vi "PAQmem_constructor.vi"(8 "error in (no error)":errorcluster, 9 "TAGs":string[](array[string]), 10 "LayerInfo":T1, 11 "PAQ-memory in":refnum<class "PAQ-memory.lvclass">) -> (0 "error out":errorcluster, 3 "PAQ-memory out":refnum<class "PAQ-memory.lvclass">)   [LabVIEW 2020, in "Sgraph_lib_V1.lvlib" / "PAQ-memory.lvclass"]
uses:
  PAQ-memory.lvclass
  PAQ-memory.lvclass/PAQ-memory.ctl
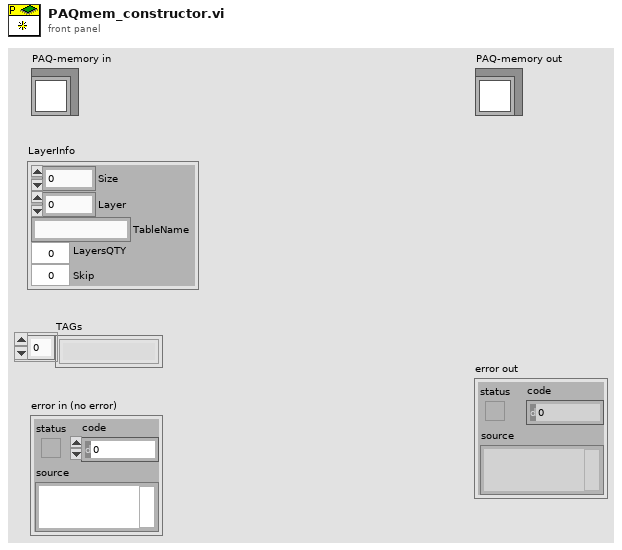
[diagram p1: front panel]
types:
  T1 = cluster{"Size":i32, "Layer":i32, "TableName":string, "LayersQTY":i32, "Skip":i32}
  T2 = cluster{"source":refnum<data-value>, "status":refnum<data-value>, "data":refnum<data-value>, "max":refnum<data-value>, "min":refnum<data-value>}
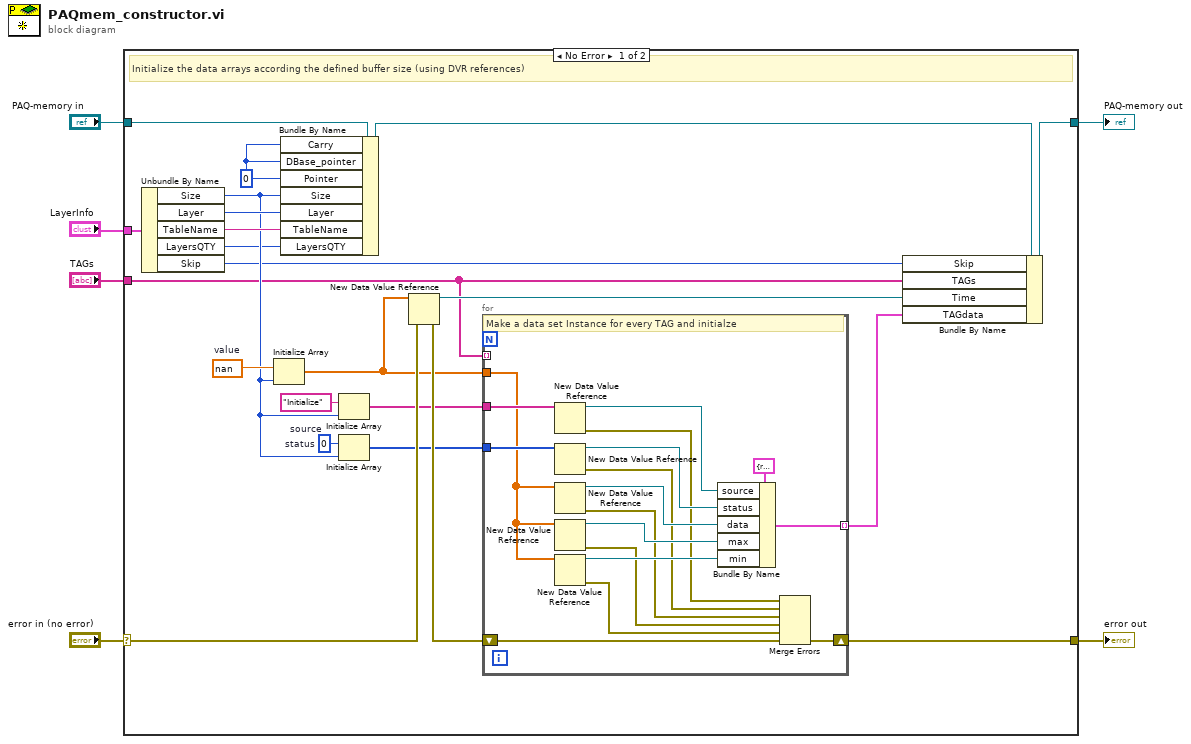
[diagram p0: block diagram]
diagram:
  n1 = case shown="No Error" "error in (no error)" {
    selector: "error in (no error)" -> [w18 w47]
    tunnel: [w15 w47] -> w1
    tunnel: [w19 w46] -> w2
    tunnel: "PAQ-memory in" -> [w25 w46]
    tunnel: "LayerInfo" -> [w28 _]
    tunnel: "TAGs" -> [w14 _]
    frame No Error {
      w21 = nan  # value
      w22 = u32 0  # status
      w23 = "Initialize"  # source
      w8 = 0 ("Pointer")
      # "Initialize the data arrays according the defined buffer size (using DVR references)"
      n2 = Unbundle By Name(w28) -> ("Size"=w17:i32, "Layer"=w27:i32, "TableName"=w26:string, "LayersQTY"=w13:i32, "Skip"=w7:i32)
      n3 = Initialize Array(w21, w17) -> (w12:dbl[])
      n4 = Bundle By Name(cluster=w25, "Carry"=w8, "DBase_pointer"=w8, "Pointer"=w8, "Size"=w17, "Layer"=w27, "TableName"=w26, "LayersQTY"=w13) -> (w24:refnum<class "PAQ-memory.lvclass">)
      n5 = Initialize Array(w23, w17) -> (w11:string[])
      n6 = Initialize Array(w22, w17) -> (w9:u32[])
      n7 = New Data Value Reference(data value=w12, error in=w18) -> (data value reference=w20:refnum<data-value>, error out=w16:errorcluster)
      n8 = for {
        tunnel: w12 -> [w38]
        tunnel: w11 -> [w40]
        shift-right: [w29] -> w15
        shift-left: w16 -> [w30]
        tunnel: w9 -> [w39]
        tunnel: [w36] -> w10 mode=indexing
        tunnel: w14 -> [_] mode=indexing
        # "Make a data set Instance for every TAG and initialze"
        n9 = New Data Value Reference(data value=w40) -> (data value reference=w45:refnum<data-value>, error out=w35:errorcluster)  [unwired: 1 in]
        n10 = New Data Value Reference(data value=w39) -> (data value reference=w44:refnum<data-value>, error out=w34:errorcluster)  [unwired: 1 in]
        n11 = New Data Value Reference(data value=w38) -> (data value reference=w43:refnum<data-value>, error out=w33:errorcluster)  [unwired: 1 in]
        n12 = New Data Value Reference(data value=w38) -> (data value reference=w42:refnum<data-value>, error out=w32:errorcluster)  [unwired: 1 in]
        n13 = New Data Value Reference(data value=w38) -> (data value reference=w41:refnum<data-value>, error out=w31:errorcluster)  [unwired: 1 in]
        n14 = Bundle By Name(cluster=T2 {"source"=refnum, "status"=refnum, "data"=refnum, "max"=refnum, "min"=refnum} ("TAGdata"), "source"=w45, "status"=w44, "data"=w43, "max"=w42, "min"=w41) -> (w36:T2)
        n15 = Merge Errors(w35, w34, w33, w32, w31, w30) -> (w29:errorcluster)
      }
      n16 = Bundle By Name(cluster=w24, "Skip"=w7, "TAGs"=w14, "Time"=w20, "TAGdata"=w10) -> (w19:refnum<class "PAQ-memory.lvclass">)
    }
    frame Error {
      # "If error then empty all arrays"
    }
  }
  "error out" <- w1
  "PAQ-memory out" <- w2
